vi "view deploy screen.vi"(8 "error in":errorcluster, 11 "deployment configuration":T2[](array[typedef])) -> (0 "error out":errorcluster)   [LabVIEW 2014, in "PL Framework Configuration Tool.lvlib"]
uses:
  PL Framework Configuration Tool.lvlib
  deployment configuration.ctl
  Framework Configuration Classes/target configuration/PL_Target Configuration.lvclass
  Classes/TBM Configuration Node/deployment configuration.ctl
  Classes/TBM Configuration Node/TBM Configuration Node.lvclass
  <vilib>/NI/DCAF UI Toolkit/Controls/Export.ctl
  Framework Configuration Classes/target configuration/PL_Target Configuration.lvclass/PL_Target Configuration.ctl
  Classes/Deployment Helpers/SCP File Transfer/SCP File Transfer.lvclass
  <vilib>/NI/RT Management/classes/FTP/FTP.lvclass
  Framework Configuration Classes/target configuration/Read name.vi
  Framework Configuration Classes/target configuration/Read hostname.vi
  Framework Configuration Classes/target configuration/Read OS.vi
  <vilib>/NI/Configuration Framework/serializable configuration/get alias.vi
  <vilib>/NI/RT Management/classes/File Transfer Behavior/File Transfer Behavior.lvclass
  <vilib>/NI/DCAF UI Toolkit/Controls/DCAF UI Elements.lvlib
panel:
  out "Deploy output":string
  in  "Deploy Errors?":bool=TRUE
  in  "Password":string
  in  "Username":string="admin"
  in  "deploy":T1
  in  "Target Destination Path":i32(listbox)
  in  "Targets":i32(listbox)
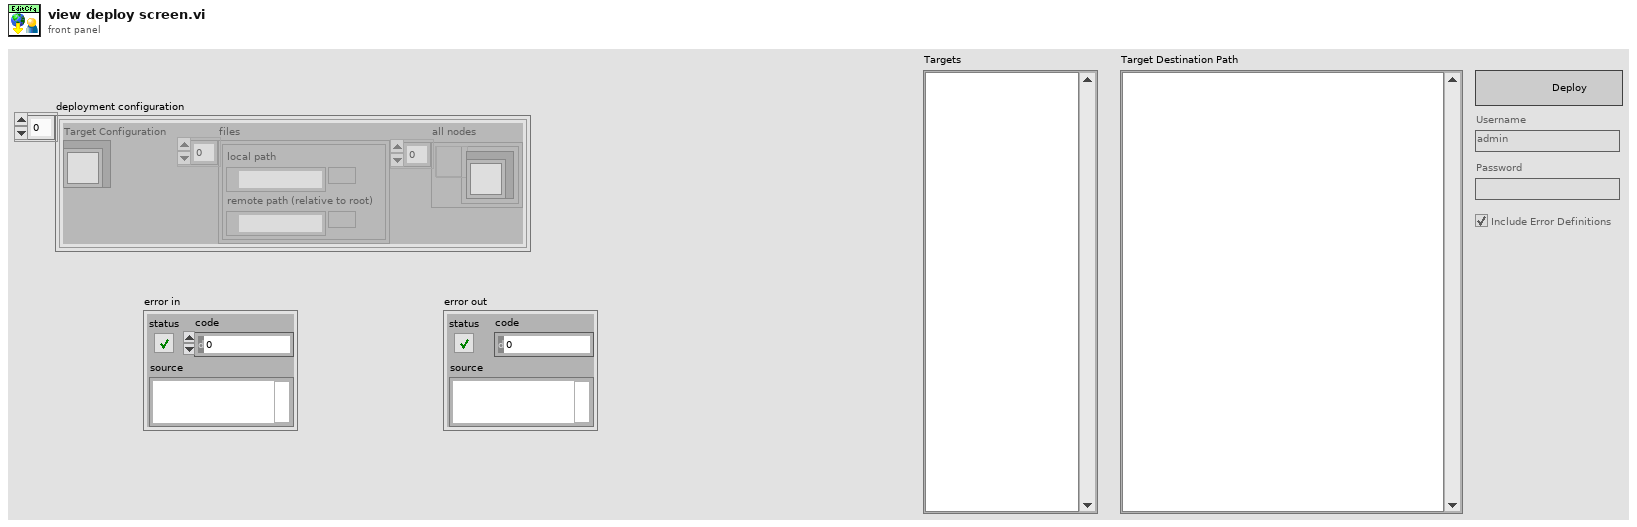
[diagram p1: front panel]
types:
  T1 = typedef "DCAF UI Elements.lvlib/Export.ctl" = bool
  T2 = typedef "PL Framework Configuration Tool.lvlib/deployment configuration.ctl" = cluster{"Target Configuration":refnum<class "PL_Target Configuration.lvclass">, "files":T3[], "all nodes":refnum<data-value>[]}
  T3 = typedef "PL Framework Configuration Tool.lvlib/TBM Configuration Node.lvclass/deployment configuration.ctl" = cluster{"local path":path, "remote path (relative to root)":path}
  T4 = enum8{"Enabled", "Disabled", "Disabled and Grayed Out"}
  T5 = typedef "TBM configuration.lvclass/Target Types.ctl" = enum16{"Windows", "Mac", "Linux", "Linux RT ARM", "VxWorks", "Pharlap", "Other", "Linux RT x64"}
  T6 = cluster{"remote path":string, "local path":path}[]
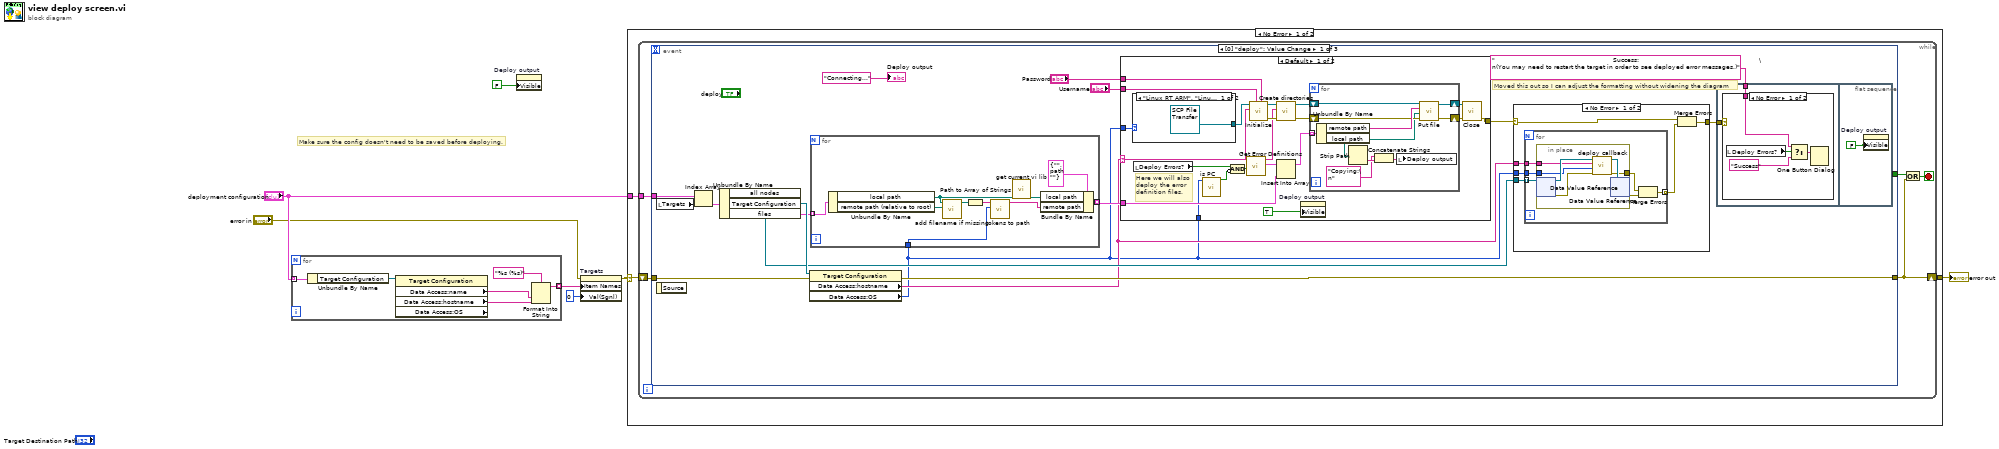
[diagram p0: block diagram]
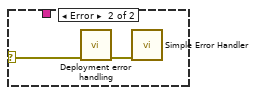
[diagram p2: hidden frame]
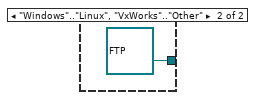
[diagram p3: hidden frame]
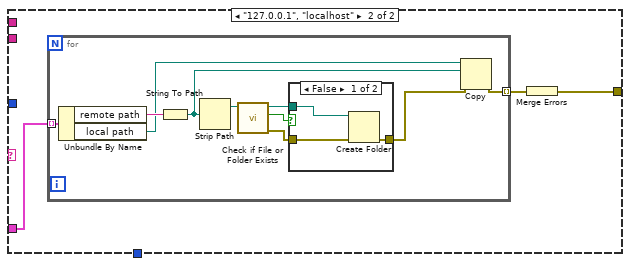
[diagram p4: hidden frame]
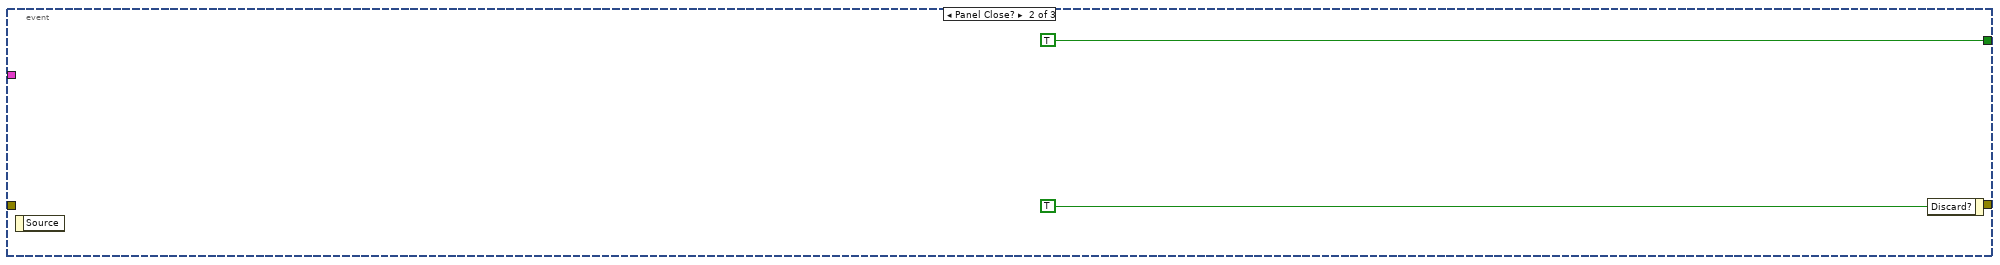
[diagram p7: hidden frame]
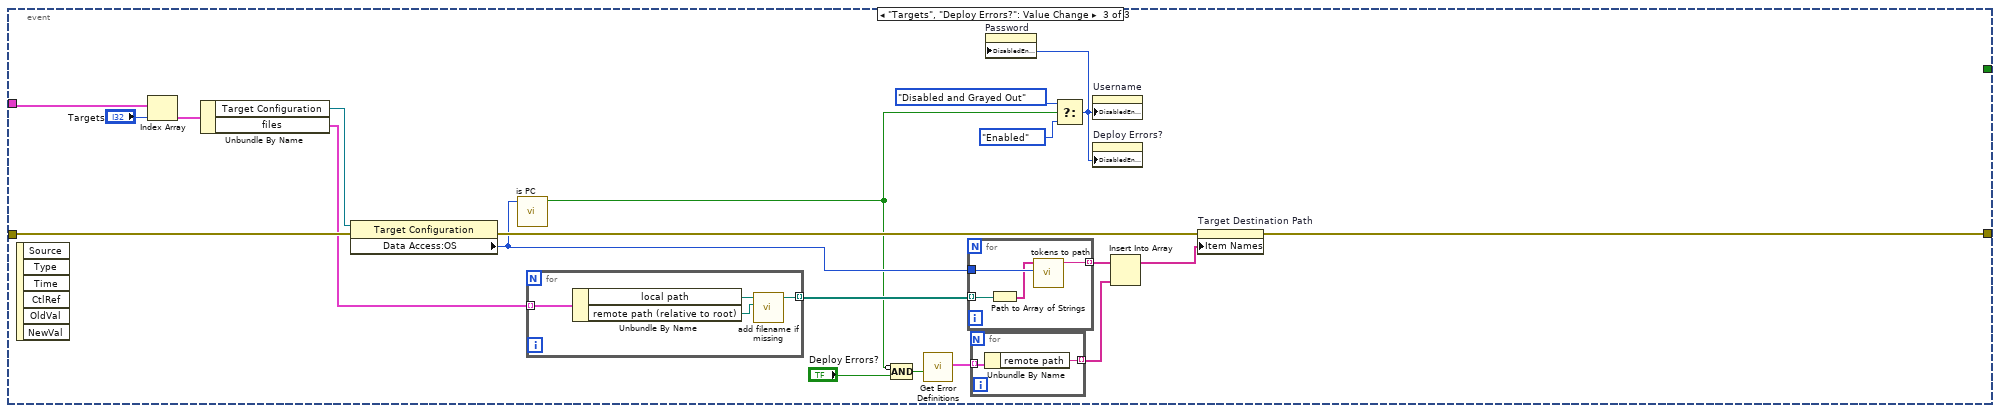
[diagram p8: hidden frame]
diagram:
  # "Make sure the config doesn't need to be saved before deploying."
  n1 = for {
    tunnel: "deployment configuration" -> [w13] mode=indexing
    tunnel: [w8] -> w7 mode=indexing
    n2 = Unbundle By Name(w13) -> ("Target Configuration"=w12:refnum<class "PL_Target Configuration.lvclass">)
    n3 = property class="Target Configuration" props=["Data Access:name", "Data Access:hostname", "Data Access:OS"](reference=w12) -> ("Data Access:name"=w11:string, "Data Access:hostname"=w10:string)  [unwired: 1 in, 3 out]
    n4 = Format Into String(format string="%s (%s)", w11, w10) -> (resulting string=w8:string)  [unwired: 2 in, 1 out]
  }
  n5 = property on="Deploy output" class="Str"("Visible"=FALSE) -> ()  [unwired: 2 in, 2 out]
  n6 = property on="Targets" class="LstBox (strict)"(error in="error in", "Item Names"=w7, "Val(Sgnl)"=0 ("Value (Signaling)")) -> (error out=w5:errorcluster)  [unwired: 1 in, 1 out]
  n7 = case shown="No Error" w5 {
    selector: w5 -> [w16 w159]
    tunnel: [w15 w159] -> w4
    tunnel: "deployment configuration" -> [w14 _]
    frame No Error {
      n8 = while {
        shift-right: [w17] -> w15
        shift-left: w16 -> [w21]
        tunnel: w14 -> [w19]
        stop <- w20 stop-if-true
        n9 = event shown="[0] \"deploy\": Value Change" {
          selector: _ -> [_ _ _]
          dyn-events: _ -> [_ _ _]
          timeout: _ -> [_ _ _]
          tunnel: [_ TRUE ("Cancel Button") _] -> w18
          tunnel: w21 -> [w26 _ w145]
          tunnel: [w34 _ w144] -> w17
          tunnel: w19 -> [w36 _ w148]
          event Value Change {
            # "Moved this out so I can adjust the formatting without widening the diagram"
            n10 = local read "Targets"() -> (w35:i32)
            n11 = event-data() -> ()  [unwired: 1 in, 1 out]
            n12 = Index Array(array=w36, index=w35) -> (element=w38:T2)
            n13 = Unbundle By Name(w38) -> ("all nodes"=w29:refnum<data-value>[], "Target Configuration"=w37:refnum<class "PL_Target Configuration.lvclass">, "files"=w25:T3[])
            n14 = property class="Target Configuration"(reference=w37, error in=w26) -> (error out=w34:errorcluster, "Data Access:hostname"=w27:string, "Data Access:OS"=w24:T5)  [unwired: 1 out]
            n15 = for {
              tunnel: w25 -> [w126] mode=indexing
              tunnel: [w124] -> w33 mode=indexing
              tunnel: w24 -> [w117]
              n16 = Unbundle By Name(w126) -> ("local path"=w119:path, "remote path (relative to root)"=w122:path)
              n17 = call "add filename if missing.vi"("remote path (relative to root)"=w122, "local path"=w119) -> ("appended path"=w121:path)  [unwired: 9 in]
              n18 = Path to Array of Strings(0:w121) -> (2:w123:string[])  [unwired: 1 out]
              n19 = call "tokens to path.vi"("Data Access:OS"=w117, "array of strings"=w123) -> ("String"=w118:string)  [unwired: 9 in]
              n20 = call "get current vi lib.vi"("Stored Path"=w119) -> ("Current VI Lib Path"=w120:path)  [unwired: 10 in]
              n21 = Bundle By Name(cluster=cluster{"remote path":string, "local path":path} {"remote path"="", "local path"=path ""} ("transfer spec"), "local path"=w120, "remote path"=w118) -> (w124:cluster{"remote path":string, "local path":path})
            }
            n22 = case shown="Default" w27 {
              selector: w27 -> [w62 _]
              tunnel: w33 -> [w53 w81]
              tunnel: w24 -> [w68 _]
              tunnel: "Username" -> [w65 _]
              tunnel: "Password" -> [w66 _]
              tunnel: [w63 w82] -> w30
              tunnel: w24 -> [w50 _]
              frame Default {
                # "Here we will also \ndeploy the error \ndefinition files."
                n23 = case shown="\"Linux RT ARM\", \"Linux RT x64\"" w68 {
                  tunnel: [refnum<class "SCP File Transfer.lvclass"> refnum ("Tag Editor Core:SCP File Transfer.lvclass") refnum<class "FTP.lvclass"> refnum ("FTP in")] -> w67
                  frame "Linux RT ARM", "Linux RT x64" {
                  }
                  frame "Windows".."Linux", "VxWorks".."Other" {
                  }
                }
                n24 = local read "Deploy Errors?"() -> (w57:bool)
                n25 = call "is PC"("OS"=w50) -> ("is PC?"=w56:bool)  [unwired: 10 in]
                n26 = Compound Arithmetic op=AND(w57, invert w56) -> (w55:bool)
                n27 = call "Get Error Definitions.vi"("Deploy Errors?"=w55) -> ("Err Defs"=w54:T6, "Unique Paths"=w51:string[])  [unwired: 9 in]
                n28 = call-dynamic "Initialize.vi"("Password"=w66, "Username"=w65, "Address"=w62, "File Transfer Behavior in"=w67) -> ("error out"=w60:errorcluster, "File Transfer Behavior out"=w61:refnum<class "File Transfer Behavior.lvclass">)  [unwired: 6 in]
                n29 = call <vilib>:"Create directories.vi"("error in (no error)"=w60, "Directories to create"=w51, "File Transfer Behavior in"=w61) -> ("error out"=w58:errorcluster, "File Transfer Behavior out"=w59:refnum<class "File Transfer Behavior.lvclass">)  [unwired: 6 in, 1 out]
                n30 = Insert Into Array(array=w54, new element=w53) -> (w52:T6)  [unwired: 1 in]
                n31 = property on="Deploy output" class="Str"("Visible"=TRUE) -> ()  [unwired: 2 in, 2 out]
                n32 = for {
                  shift-right: [w78] -> w64
                  shift-left: w59 -> [w75]
                  shift-right: [w76] -> w49
                  shift-left: w58 -> [w73]
                  tunnel: w52 -> [w77] mode=indexing
                  n33 = Unbundle By Name(w77) -> ("remote path"=w74:string, "local path"=w72:path)
                  n34 = Strip Path(path=w72) -> (name=w70:string)  [unwired: 1 out]
                  n35 = Concatenate Strings("Copying:\n" ("Deploy output"), w70) -> (w71:string)
                  n36 = local write "Deploy output"(w71) -> ()
                  n37 = call-dynamic "Put file.vi"("error in (no error)"=w73, "Local path"=w72, "Remote path"=w74, "File Transfer Behavior in"=w75) -> ("error out"=w76:errorcluster, "File Transfer Behavior out"=w78:refnum<class "File Transfer Behavior.lvclass">)  [unwired: 6 in]
                }
                n38 = call-dynamic "Close.vi"("error in (no error)"=w49, "File Transfer Behavior in"=w64) -> ("error out"=w63:errorcluster)  [unwired: 9 in]
              }
              frame "127.0.0.1", "localhost" {
                n39 = for {
                  tunnel: [w92] -> w83 mode=indexing
                  tunnel: w81 -> [w93] mode=indexing
                  n40 = Unbundle By Name(w93) -> ("remote path"=w91:string, "local path"=w85:path)
                  n41 = String To Path(string=w91) -> (path=w84:path)
                  n42 = Strip Path(path=w84) -> (stripped path=w89:path)  [unwired: 1 out]
                  n43 = call <vilib>:"Check if File or Folder Exists.vi"("path"=w89) -> ("error out"=w87:errorcluster, "file or folder exists?"=w88:bool, "dup path"=w90:path)  [unwired: 8 in]
                  n44 = case shown="False" w88 {
                    tunnel: w90 -> [w96 _]
                    tunnel: w87 -> [w95 w97]
                    tunnel: [w94 w97] -> w86
                    frame False {
                      n45 = Create Folder(path (use dialog)=w96, error in=w95) -> (error out=w94:errorcluster)  [unwired: 1 in, 2 out]
                    }
                    frame True {
                    }
                  }
                  n46 = Copy(8:w86, 10:w84, 11:w85) -> (0:w92:errorcluster)  [unwired: 2 in, 2 out]
                }
                n47 = Merge Errors(w83) -> (w82:errorcluster)
              }
            }
            n48 = case shown="No Error" w30 {
              selector: w30 -> [w100 w116]
              tunnel: w29 -> [w103 _]
              tunnel: [w102 w116] -> w28
              tunnel: w27 -> [w99 _]
              tunnel: w24 -> [w98 _]
              frame No Error {
                n49 = for {
                  tunnel: w103 -> [w109] mode=indexing
                  tunnel: [w108] -> w101 mode=indexing
                  tunnel: w99 -> [w105]
                  tunnel: w98 -> [w104]
                  n50 = in-place {
                    in-place-border: [w113] -> w106
                    in-place-border: w105 -> [w111]
                    in-place-border: w104 -> [w110]
                    n51 = in-place-dvr #1(w109) -> (w115:refnum<class "TBM Configuration Node.lvclass">, w112:errorcluster)
                    n52 = call-dynamic "deploy callback.vi"("error in"=w112, "Target Types"=w110, "IP"=w111, "TBM Configuration Node in"=w115) -> ("error out"=w113:errorcluster, "TBM Configuration Node out"=w114:refnum<class "TBM Configuration Node.lvclass">)  [unwired: 6 in]
                    n53 = in-place-dvr #1(w114) -> (w107:errorcluster)  [unwired: 1 out]
                  }
                  n54 = Merge Errors(w106, w107) -> (w108:errorcluster)
                }
                n55 = Merge Errors(w100, w101) -> (w102:errorcluster)
              }
              frame Error {
              }
            }
            n56 = flat-sequence {
              tunnel: w28 -> [w40]
              tunnel: "                                                           Success:                                                            \n(You may need to restart the target in order to see deployed error messages.)" ("message") -> [w39]
              frame #0 {
                n57 = case shown="No Error" w40 {
                  selector: w40 -> [_ w45]
                  tunnel: w39 -> [w41 _]
                  frame No Error {
                    n58 = local read "Deploy Errors?"() -> (w42:bool)
                    n59 = Select(t=w41, s=w42, f="Success" ("message")) -> (s? t:f=w44:string)
                    n60 = One Button Dialog(message=w44) -> ()  [unwired: 1 in, 1 out]
                  }
                  frame Error {
                    n61 = call "Deployment error handling.vi"("error in (no error)"=w45) -> ("error out"=w46:errorcluster)  [unwired: 10 in]
                    n62 = call <vilib>:"Simple Error Handler.vi"("error in (no error)"=w46) -> ()  [unwired: 4 in, 5 out]
                  }
                }
              }
              frame #1 {
                n63 = property on="Deploy output" class="Str"("Visible"=FALSE) -> ()  [unwired: 2 in, 2 out]
              }
            }
            "Deploy output" <- "Connecting..." ("Deploy output")
          }
          event Panel Close? {
            n64 = event-data() -> ()  [unwired: 1 in, 1 out]
            n65 = event-data("Discard?"=TRUE) -> ()  [unwired: 1 in, 1 out]
          }
          event "Targets", "Deploy Errors?": Value Change {
            n66 = event-data() -> ()  [unwired: 1 in, 6 out]
            n67 = Index Array(array=w148, index="Targets") -> (element=w146:T2)
            n68 = Unbundle By Name(w146) -> ("Target Configuration"=w142:refnum<class "PL_Target Configuration.lvclass">, "files"=w131:T3[])
            n69 = property class="Target Configuration"(reference=w142, error in=w145) -> (error out=w143:errorcluster, "Data Access:OS"=w137:T5)  [unwired: 1 out]
            n70 = call "is PC"("OS"=w137) -> ("is PC?"=w135:bool)  [unwired: 10 in]
            n71 = for {
              tunnel: w131 -> [w158] mode=indexing
              tunnel: [w155] -> w141 mode=indexing
              n72 = Unbundle By Name(w158) -> ("local path"=w157:path, "remote path (relative to root)"=w156:path)
              n73 = call "add filename if missing.vi"("remote path (relative to root)"=w156, "local path"=w157) -> ("appended path"=w155:path)  [unwired: 9 in]
            }
            n74 = Compound Arithmetic op=AND(invert w135, "Deploy Errors?") -> (w136:bool)
            n75 = call "Get Error Definitions.vi"("Deploy Errors?"=w136) -> ("Err Defs"=w133:T6)  [unwired: 9 in, 1 out]
            n76 = for {
              tunnel: w141 -> [w154] mode=indexing
              tunnel: w137 -> [w153]
              tunnel: [w152] -> w130 mode=indexing
              n77 = Path to Array of Strings(0:w154) -> (2:w151:string[])  [unwired: 1 out]
              n78 = call "tokens to path.vi"("Data Access:OS"=w153, "array of strings"=w151) -> ("String"=w152:string)  [unwired: 9 in]
            }
            n79 = for {
              tunnel: w133 -> [w150] mode=indexing
              tunnel: [w149] -> w132 mode=indexing
              n80 = Unbundle By Name(w150) -> ("remote path"=w149:string)
            }
            n81 = Select(t=T4."Disabled and Grayed Out" ("Disabled"), s=w135, f=T4."Enabled") -> (s? t:f=w138:T4)
            n82 = property on="Password" class="Str"("DisabledEnum"=w138) -> ()  [unwired: 2 in, 2 out]
            n83 = property on="Username" class="Str"("DisabledEnum"=w138) -> ()  [unwired: 2 in, 2 out]
            n84 = property on="Deploy Errors?" class="Bool (strict)"("DisabledEnum"=w138) -> ()  [unwired: 2 in, 2 out]
            n85 = Insert Into Array(array=w130, new element=w132) -> (w129:string[])  [unwired: 1 in]
            n86 = property on="Target Destination Path" class="LstBox (strict)"(error in=w143, "Item Names"=w129) -> (error out=w144:errorcluster)  [unwired: 1 in, 1 out]
          }
        }
        n87 = Or(x=w18, y=w17) -> (x .or. y?=w20:bool)
      }
    }
    frame Error {
    }
  }
  "error out" <- w4
